vi "RT_Status_Publish.vi"(8 "error in (no error)":errorcluster={"status"=FALSE, "code"=0, "source"="\"\""}, 10 "samples":string, 11 "Controller statuses":string) -> (0 "error out":errorcluster={"status"=FALSE, "code"=0, "source"="\"\""}, 2 "status ok":bool, 3 "Registry messages":string)   [LabVIEW 2026]
doc: "INTENT: Share controller/IO health and feedback. LOGIC: Publish bounded updates with timestamps into registry/transport service."
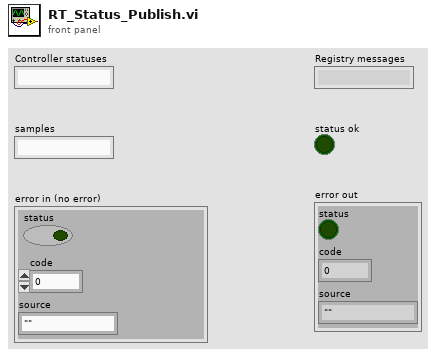
[diagram p1: front panel]
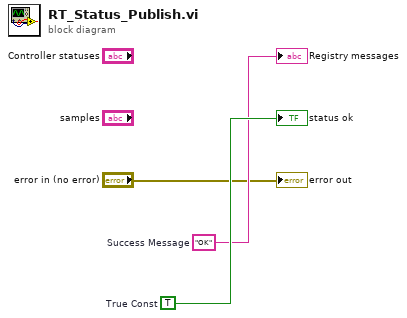
[diagram p0: block diagram]
diagram:
  w3 = TRUE  # True Const
  w2 = "OK"  # Success Message
  "Registry messages" <- w2
  "status ok" <- w3
  "error out" <- "error in (no error)"
